vi "Export.vi"(8 "error in (no error)":errorcluster, 11 "Test Report in":refnum<class "Test Report.Default.lvclass">) -> (0 "error out":errorcluster, 3 "Test Report out":refnum<class "Test Report.Default.lvclass">)   [LabVIEW 2020, in "Caraya.lvlib" / "Test Report.Default.lvclass"]
uses:
  Test Report.Default.lvclass
  C:/projects/caraya/src/classes/Test Report/Test Report.lvclass
  Test Report.Default.lvclass/Test Report.Default.ctl
  Test Report/Test Report.lvclass
  Test Result/Test Result.lvclass
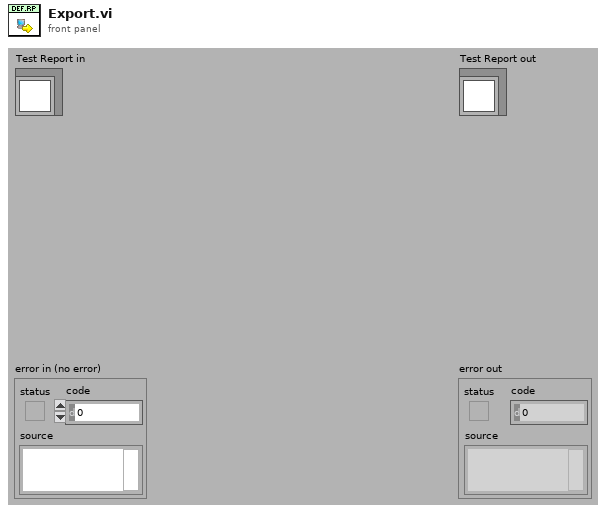
[diagram p1: front panel]
types:
  T1 = enum16{"open", "replace", "create", "open or create", "replace or create", "replace or create with confirmation"}
  T2 = typedef "Caraya.lvlib/Test Result.lvclass/Node Results (Extended).ctl" = cluster{"Test Node":T3, "Assertions":T5[]}
  T3 = typedef "Caraya.lvlib/Test Result.lvclass/Test Node (Extended).ctl" = cluster{"Test Registration":T4, "Defined":bool, "Passed":bool, "properties":variant}
  T4 = typedef "Caraya.lvlib/Test Result.lvclass/Test Registration Data.ctl" = cluster{"Name":string, "Call Chain":string[], "Time Stamp":timestamp, "Test ID":string, "Caller ID":string}
  T5 = typedef "Caraya.lvlib/Test Result.lvclass/Assert Event Data (Extended).ctl" = cluster{"name":string, "passed":bool, "call-chain":string[], "test-error":errorcluster, "timestamp":timestamp, "assert-id":string, "test-id":string, "time":dbl, "message":string, "properties":variant, "measurements":variant, "user-defined":variant}
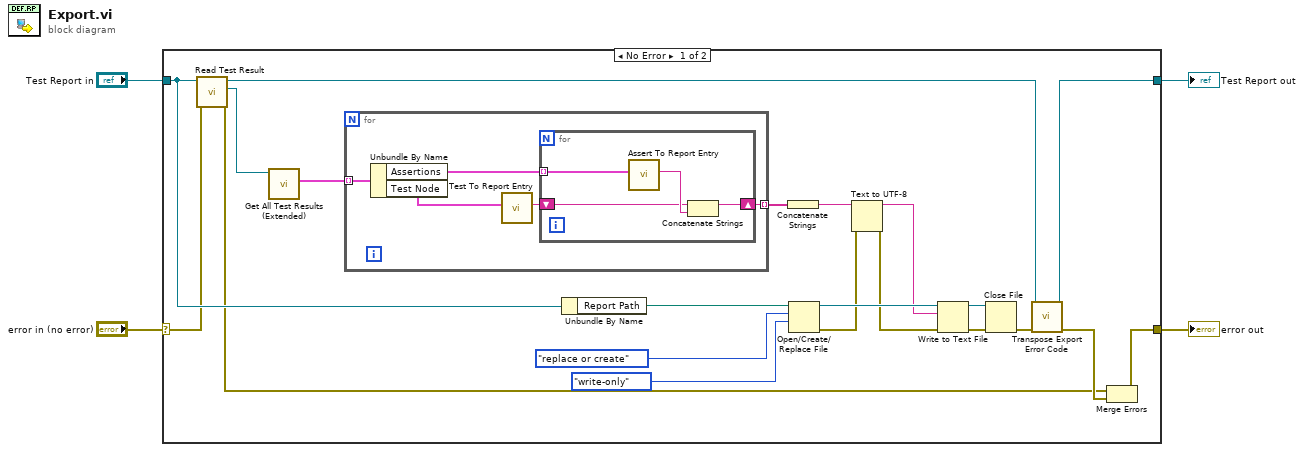
[diagram p0: block diagram]
diagram:
  n1 = case shown="No Error" "error in (no error)" {
    selector: "error in (no error)" -> [w18 w36]
    tunnel: [w13 w36] -> w3
    tunnel: [w9 w35] -> w1
    tunnel: "Test Report in" -> [w19 w35]
    frame No Error {
      n2 = call "Read Test Result.vi"("error in (no error)"=w18, "Test Report in"=w19) -> ("error out"=w12:errorcluster, "Caraya.lvlib:Test Result.lvclass"=w17:refnum<class "Test Result.lvclass">, "Test Report out"=w10:refnum<class "Test Report.Default.lvclass">)  [unwired: 7 in]
      n3 = call "Get All Test Results (Extended).vi"("Test Result in"=w17) -> ("Test Results"=w16:T2[])  [unwired: 8 in, 2 out]
      n4 = for {
        tunnel: w16 -> [w29] mode=indexing
        tunnel: [w28] -> w15 mode=indexing
        n5 = Unbundle By Name(w29) -> ("Assertions"=w27:T5[], "Test Node"=w26:T3)
        n6 = call "Test To Report Entry.vi"("Test Node"=w26) -> ("String"=w30:string)  [unwired: 9 in, 1 out]
        n7 = for {
          shift-right: [w32] -> w28
          shift-left: w30 -> [w33]
          tunnel: w27 -> [w31] mode=indexing
          n8 = call "Assert To Report Entry.vi"("Assert Event Data"=w31) -> ("String"=w34:string)  [unwired: 9 in, 1 out]
          n9 = Concatenate Strings(w33, w34) -> (w32:string)
        }
      }
      n10 = Unbundle By Name(w19) -> ("Report Path"=w20:path)
      n11 = Concatenate Strings(w15) -> (w8:string)
      n12 = Open/Create/Replace File(file path (use dialog)=w20, operation (0:open)=T1."replace or create", access (0:read/write)=enum16{"read/write", "read-only", "write-only"}."write-only") -> (refnum out=w23:refnum<file>, error out=w6:errorcluster)  [unwired: 3 in, 1 out]
      n13 = Text to UTF-8(8:w6, 11:w8) -> (0:w5:errorcluster, 3:w7:string)  [unwired: 1 in]
      n14 = Write to Text File(file (use dialog)=w23, text=w7, error in=w5) -> (refnum out=w22:refnum<file>, error out=w21:errorcluster)  [unwired: 1 in, 1 out]
      n15 = Close File(refnum=w22, error in=w21) -> (error out=w11:errorcluster)  [unwired: 1 out]
      n16 = call-dynamic "Transpose Export Error Code.vi"("error in (no error)"=w11, "Test Report"=w10) -> ("error out"=w14:errorcluster, "Test Report out"=w9:refnum<class "Test Report.Default.lvclass">)  [unwired: 8 in]
      n17 = Merge Errors(w12, w14) -> (w13:errorcluster)
    }
    frame Error {
    }
  }
  "error out" <- w3
  "Test Report out" <- w1
